vi "CRC.vi"(11 "Data":string) -> (0 "CRCL":string, 1 "CRCH":string, 2 "CRC16":string, 3 "Data+CRC":string)   [LabVIEW 2025, in "Procotol_class.lvclass"]
uses:
  Procotol_class.lvclass
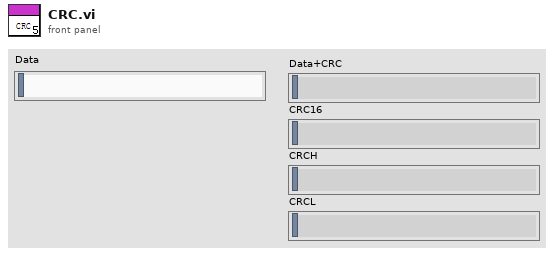
[diagram p1: front panel]
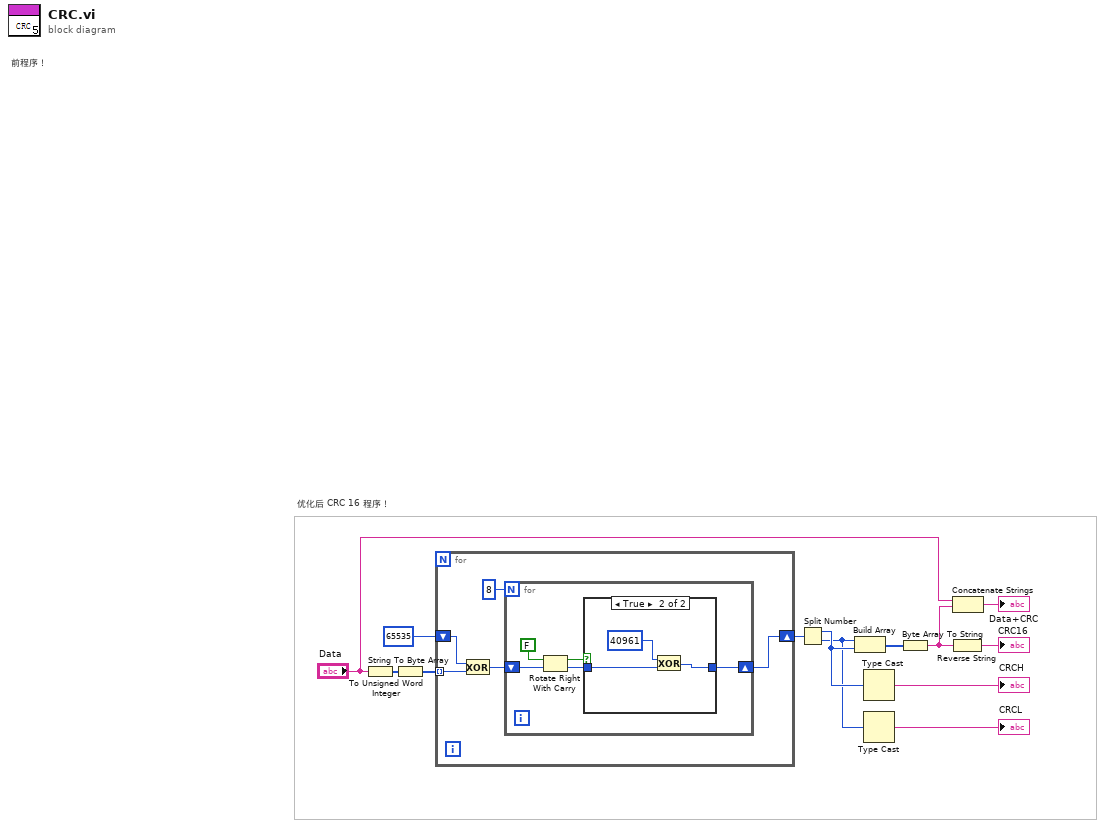
[diagram p0: block diagram]
diagram:
  # "优化后 CRC 16 程序！"
  # "前程序！"
  n1 = String To Byte Array(string="Data") -> (unsigned byte array=w11:u8[])
  n2 = To Unsigned Word Integer(number=w11) -> (unsigned 16bit integer=w10:u16[])
  n3 = for {
    shift-right: [w15] -> w12
    shift-left: u16 65535 -> [w16]
    tunnel: w10 -> [w14] mode=indexing
    n4 = Exclusive Or(1:w14, 2:w16) -> (0:w17:u16)
    n5 = for {
      N: 8 -> [_]
      shift-right: [w22] -> w15
      shift-left: w17 -> [w21]
      n6 = Rotate Right With Carry ("带进位的右移位")(2:w21, 3:FALSE ("Übertrag")) -> (0:w23:u16, 1:w20:bool)
      n7 = case shown="True" w20 {
        tunnel: w23 -> [w24 w26]
        tunnel: [w24 w25] -> w22
        frame False {
        }
        frame True {
          n8 = Exclusive Or(1:w26, 2:u16 40961) -> (0:w25:u16)
        }
      }
    }
  }
  n9 = Split Number(x=w12) -> (hi(x)=w5:u8, lo(x)=w2:u8)
  n10 = Build Array(w2, w5) -> (w9:u8[])
  n11 = Type Cast(x=w5) -> (*(type *) &x=→"CRCH":string)  [unwired: 1 in]
  n12 = Type Cast(x=w2) -> (*(type *) &x=→"CRCL":string)  [unwired: 1 in]
  n13 = Byte Array To String(unsigned byte array=w9) -> (string=w7:string)
  n14 = Reverse String(1:w7) -> (0:→"CRC16":string)
  n15 = Concatenate Strings("Data", w7) -> (→"Data+CRC":string)
